vi "OpenGDS_Installer.vi"() -> ()   [LabVIEW 2020]
uses:
  OpenGDS_Installer_State.ctl
  <vilib>/Utility/config.llb/Read Key (String).vi
  <vilib>/zip/NI_Unzip.lvlib
  <vilib>/Utility/config.llb/NI_LVConfig.lvlib
panel:
  out "Tab":enum32{"Full", "Small"}(tab)
  in  "Restart":bool
  out "FullDetailsText":string
  out "FullHeader":string
  out "SmallDetailsText":string
  out "SmallHeaderText":string
  out "SmallSteps":T1(tab)
  in  "Accept":bool
  out "Lic":string
  in  "RemoveCompCode_OpenGDSSource":bool
  in  "RemoveCompCode_AddVis":bool
  out "Ready?-Text":string
  out "Status:":u8(slide) caption="Removing files" scale=0.0..100.0
  out "ProgressText":string
  in  "Back":bool
  in  "Next":bool
  in  "Cancel":bool
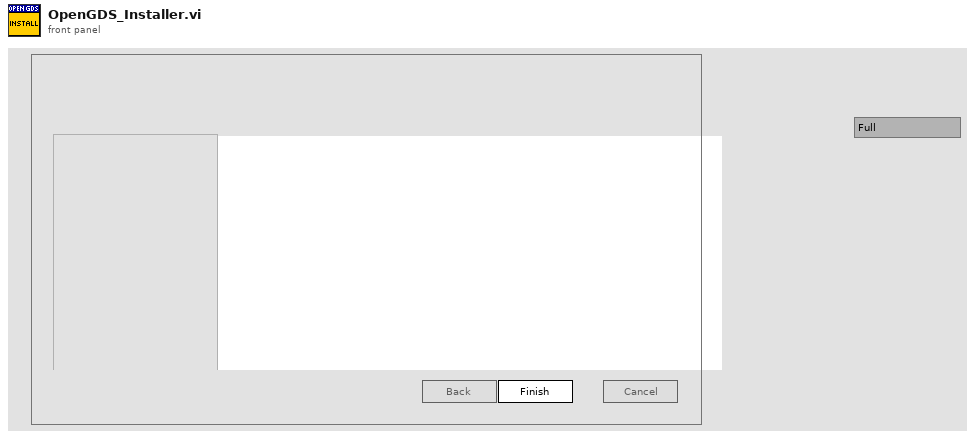
[diagram p1: front panel]
types:
  T1 = enum32{"License", "Options", "Ready?", "Progress"}
  T2 = typedef "OpenGDS_Installer_State.ctl" = enum16{"Init", "License", "Options", "Ready?", "Progress", "Cancelled", "Finished"}
  T3 = cluster{"State":T2, "FilesCopied":i32, "ErrorTest":string, "Files":path[], "ReCompile":bool, "RemoveCC":bool[]}
  T4 = typedef "LVRectTypeDef.ctl" = cluster{"Left":i16, "Top":i16, "Right":i16, "Bottom":i16}
  T5 = enum8{"Enabled", "Disabled", "Disabled and Grayed Out"}
  T6 = typedef "NI_LVConfig.lvlib/Config Data RefNum.ctl" = refnum<k1>
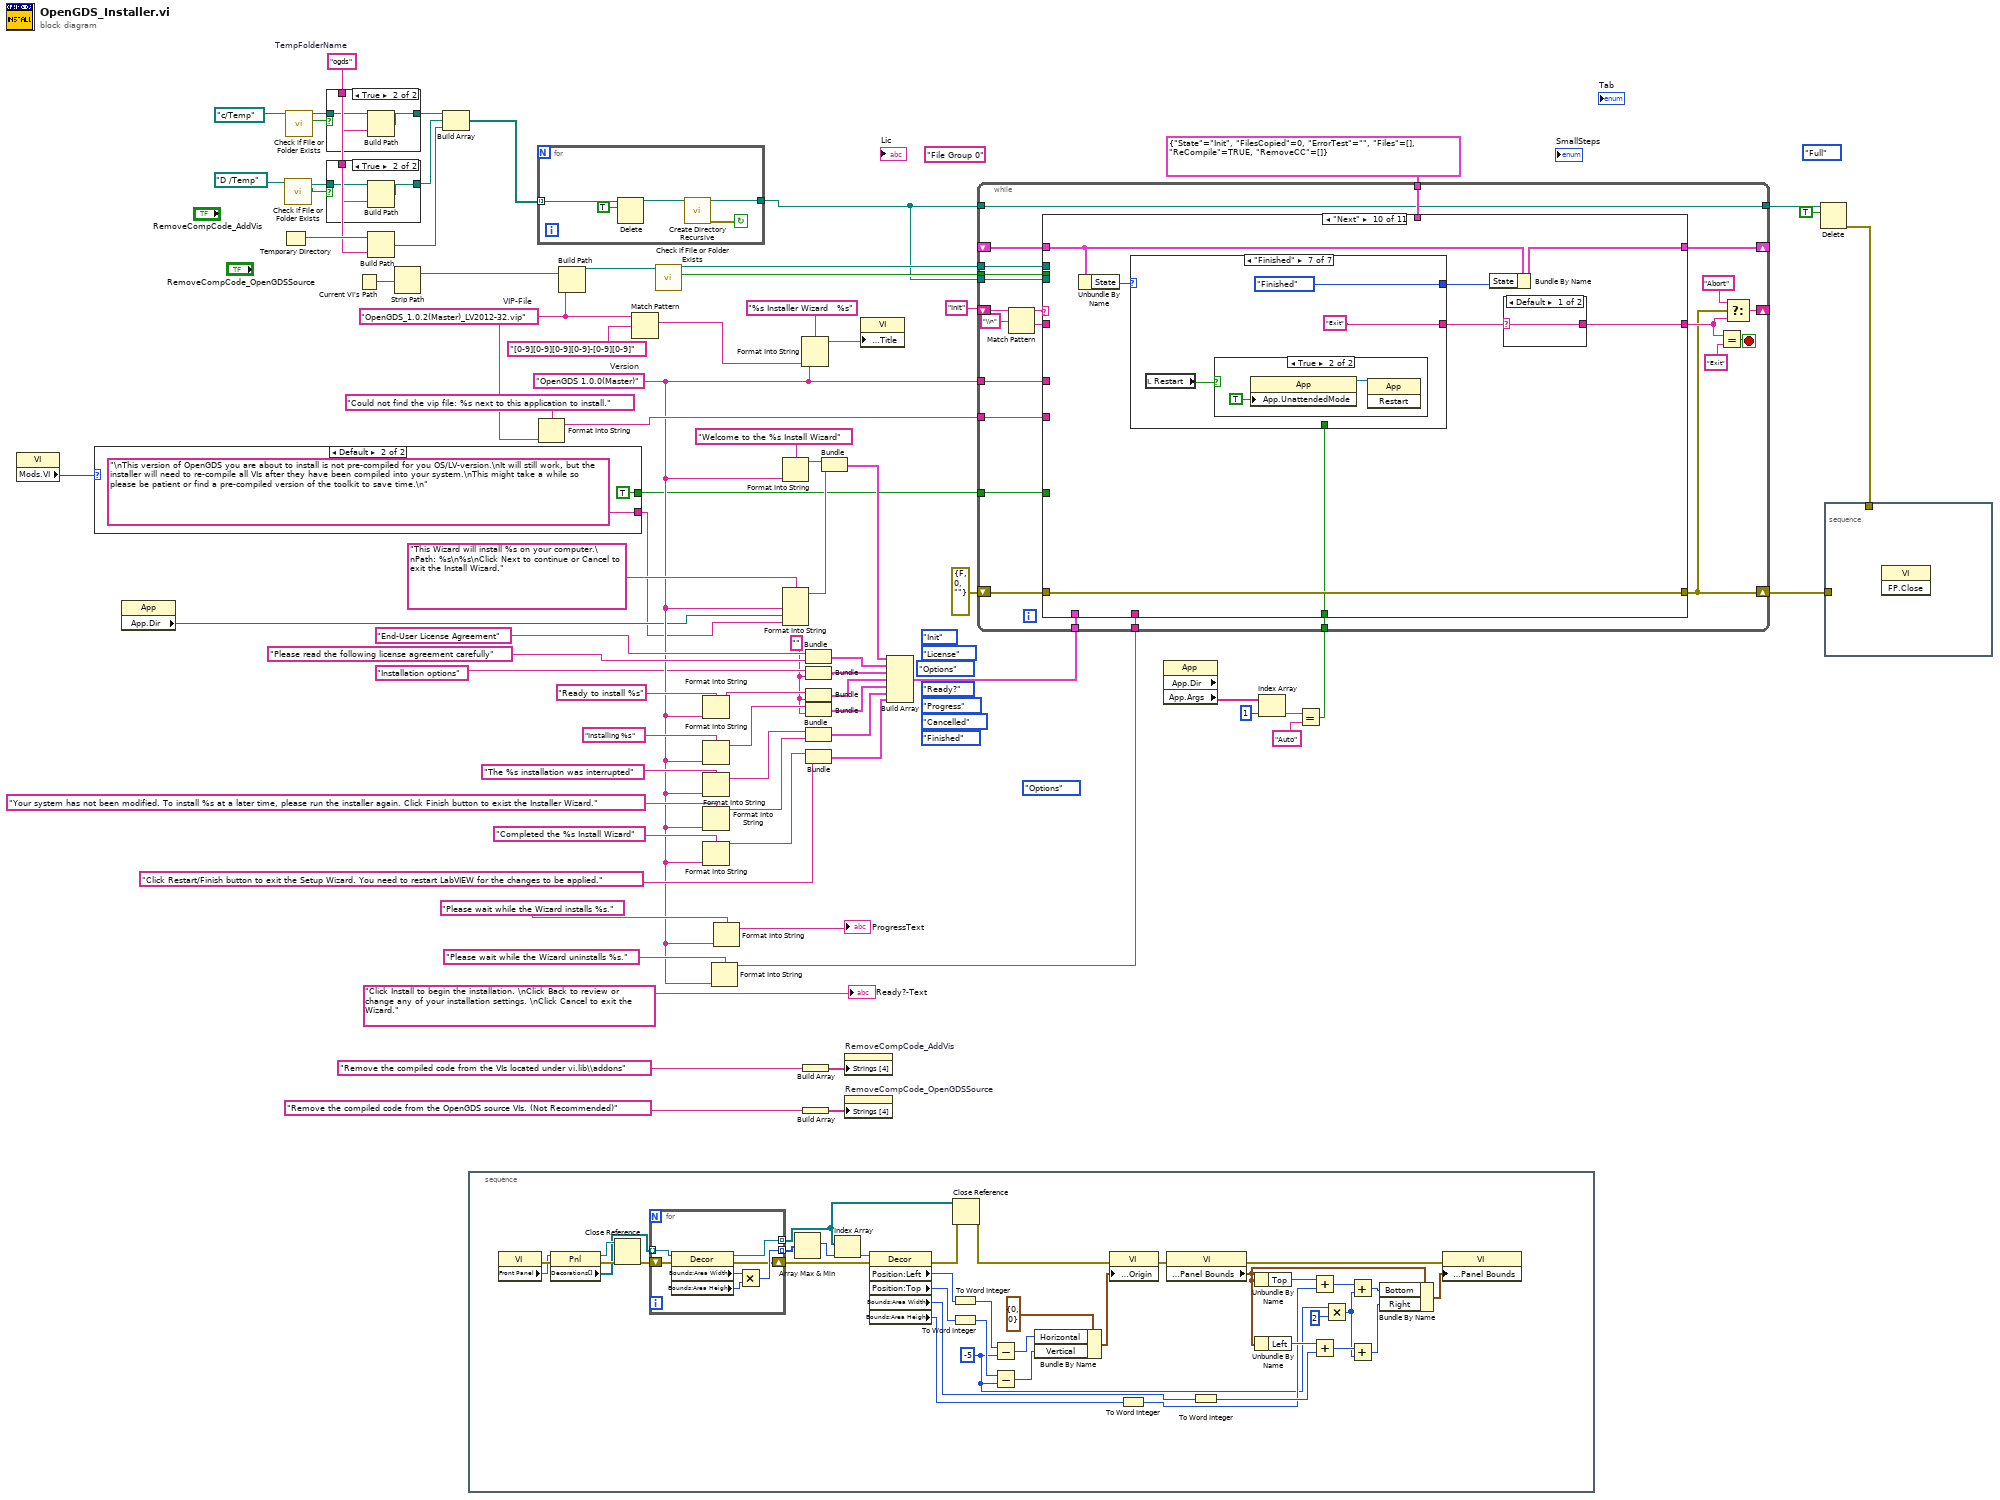
[diagram p0: block diagram]
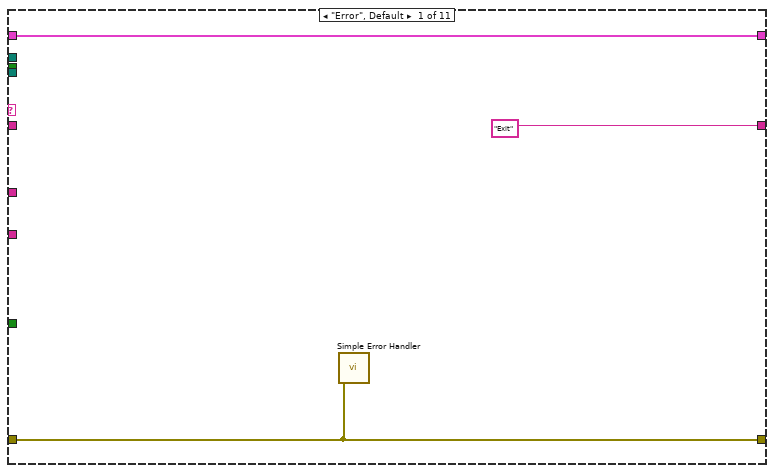
[diagram p5: hidden frame]
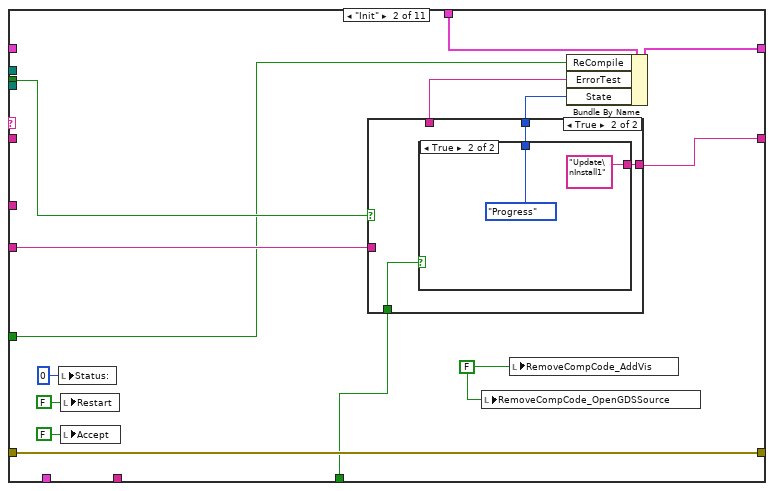
[diagram p6: hidden frame]
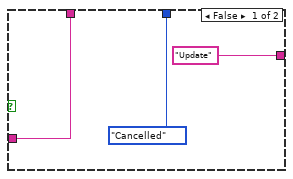
[diagram p7: hidden frame]
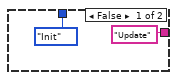
[diagram p8: hidden frame]
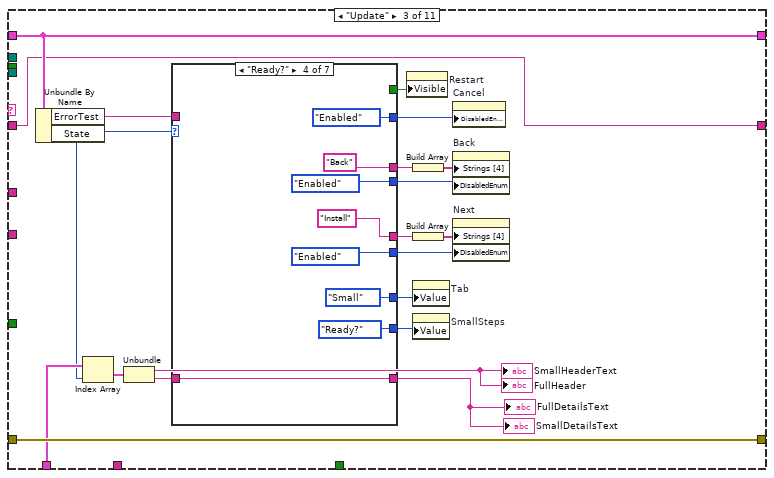
[diagram p9: hidden frame]
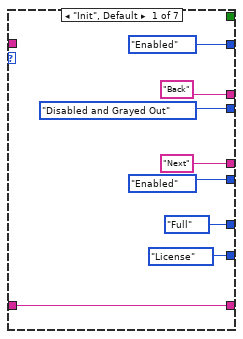
[diagram p10: hidden frame]
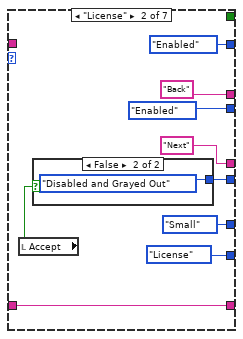
[diagram p11: hidden frame]
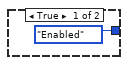
[diagram p12: hidden frame]
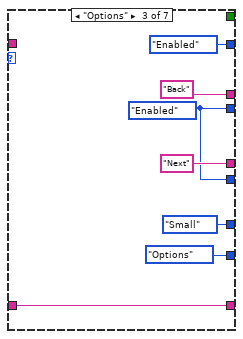
[diagram p13: hidden frame]
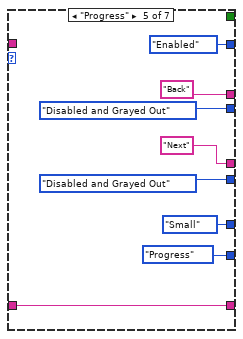
[diagram p14: hidden frame]
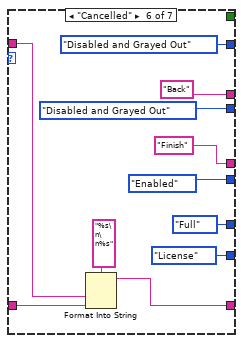
[diagram p15: hidden frame]
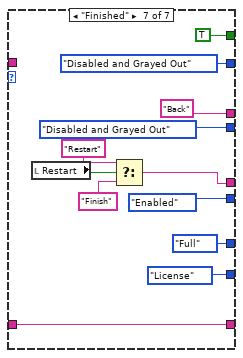
[diagram p16: hidden frame]
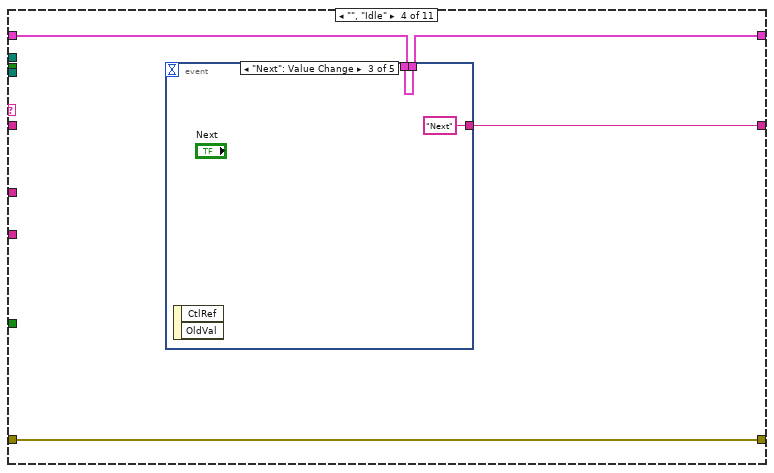
[diagram p17: hidden frame]
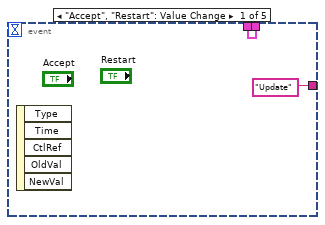
[diagram p18: hidden frame]
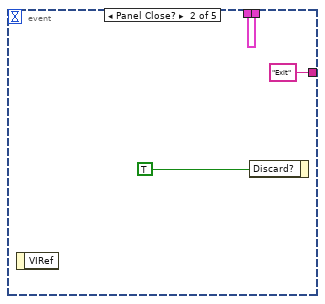
[diagram p19: hidden frame]
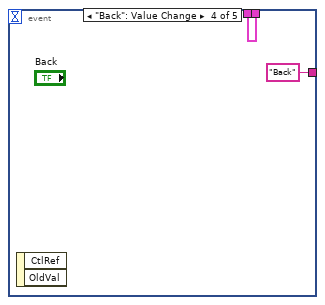
[diagram p20: hidden frame]
diagram:
  (unwired) OpenGDS_Installer_State."Options" ("State")
  (unwired) OpenGDS_Installer_State."Options" ("State")
  w17 = "ogds"  # TempFolderName
  (unwired) "File Group 0" ("section")
  w11 = "OpenGDS_1.0.2(Master)_LV2012-32.vip"  # VIP-File
  w2 = ""
  (unwired) OpenGDS_Installer_State."Finished" ("State")
  (unwired) OpenGDS_Installer_State."Cancelled" ("State")
  (unwired) OpenGDS_Installer_State."Progress" ("State")
  (unwired) OpenGDS_Installer_State."Ready?" ("State")
  (unwired) OpenGDS_Installer_State."License" ("State")
  (unwired) OpenGDS_Installer_State."Init" ("State")
  (unwired) enum32{"Full", "Small"}."Full" ("Tab")
  w40 = "OpenGDS 1.0.0(Master)"  # Version
  n1 = property class="VI"() -> ("Mods.VI"=w32:u64)  [unwired: 2 in, 2 out]
  n2 = case shown="Default" w32 {
    tunnel: [_ "\nThis version of OpenGDS you are about to install is not pre-compiled for you OS/LV-version.\nIt will still work, but the installer will need to re-compile all VIs after they have been compiled into your system.\nThis might take a while so please be patient or find a pre-compiled version of the toolkit to save time.\n"] -> w31
    tunnel: [_ TRUE] -> w30
    frame 0 {
    }
    frame Default {
    }
  }
  n3 = property class="App"() -> ("App.Dir"=w37:path)  [unwired: 2 in, 2 out]
  n4 = Temporary Directory() -> (w23:path)
  n5 = call <vilib>:"Check if File or Folder Exists.vi"("path"=path "/D /Temp") -> ("file or folder exists?"=w24:bool, "dup path"=w25:path)  [unwired: 8 in, 1 out]
  n6 = call <vilib>:"Check if File or Folder Exists.vi"("path"=path "c:/Temp") -> ("file or folder exists?"=w27:bool, "dup path"=w26:path)  [unwired: 8 in, 1 out]
  n7 = case shown="True" w27 {
    tunnel: w26 -> [w81 w84]
    tunnel: w17 -> [_ w83]
    tunnel: [w81 w82] -> w22
    frame False {
    }
    frame True {
      n8 = Build Path(base path=w84, name or relative path=w83) -> (appended path=w82:path)
    }
  }
  n9 = case shown="True" w24 {
    tunnel: w25 -> [w85 w88]
    tunnel: w17 -> [_ w87]
    tunnel: [w85 w86] -> w21
    frame False {
    }
    frame True {
      n10 = Build Path(base path=w88, name or relative path=w87) -> (appended path=w86:path)
    }
  }
  n11 = Current VI's Path() -> (path=w48:path)
  n12 = Build Path(base path=w23, name or relative path=w17) -> (appended path=w20:path)
  n13 = Strip Path(path=w48) -> (stripped path=w47:path)  [unwired: 1 out]
  n14 = Build Array(w22, w21, w20) -> (w19:path[])
  n15 = stacked-sequence {
    frame #0 {
      w92 = i16 -5 ("border spacing (2 px)")
      n16 = property on="Property Node" class="VI"() -> (error out=w125:errorcluster, "Front Panel"=w123:refnum<vi>)  [unwired: 2 in, 1 out]
      n17 = property on="Property Node" class="Pnl"(reference=w123, error in=w125) -> (reference out=w126:refnum<vi>, error out=w124:errorcluster, "Decorations[]"=w121:refnum<vi>[])
      n18 = Close Reference(reference=w126, error in (no error)=w124) -> (error out=w122:errorcluster)
      n19 = for {
        tunnel: w121 -> [w133] mode=indexing
        tunnel: [w130] -> w104 mode=indexing
        shift-right: [w128] -> w101
        shift-left: w122 -> [w129]
        tunnel: [w127] -> w91 mode=indexing
        n20 = property class="Decor"(reference=w133, error in=w129) -> (reference out=w127:refnum<vi>, error out=w128:errorcluster, "Bounds:Area Width"=w132:u32, "Bounds:Area Height"=w131:u32)
        n21 = Multiply(x=w132, y=w131) -> (x*y=w130:u32)
      }
      n22 = Array Max & Min(array=w104) -> (max index (indices)=w103:i32)  [unwired: 3 out]
      n23 = Index Array(array=w91, index=w103) -> (element=w102:refnum<vi>)
      n24 = property class="Decor"(reference=w102, error in=w101) -> (error out=w90:errorcluster, "Position:Left"=w107:i32, "Position:Top"=w110:i32, "Bounds:Area Width"=w115:u32, "Bounds:Area Height"=w113:u32)  [unwired: 1 out]
      n25 = To Word Integer(number=w107) -> (16bit integer=w94:i16)
      n26 = To Word Integer(number=w110) -> (16bit integer=w93:i16)
      n27 = Close Reference(reference=w91, error in (no error)=w90) -> (error out=w89:errorcluster)
      n28 = Subtract(x=w94, y=w92) -> (x-y=w108:i16)
      n29 = Subtract(x=w93, y=w92) -> (x-y=w109:i16)
      n30 = Bundle By Name(cluster=cluster{"Horizontal":i16, "Vertical":i16} {"Horizontal"=0, "Vertical"=0} ("Front Panel Window:Origin"), "Horizontal"=w108, "Vertical"=w109) -> (w105:cluster{"Horizontal":i16, "Vertical":i16})
      n31 = property on="Property Node" class="VI"(error in=w89, "Front Panel Window:Origin"=w105) -> (error out=w99:errorcluster)  [unwired: 1 in, 1 out]
      n32 = To Word Integer(number=w113) -> (16bit integer=w95:i16)
      n33 = property on="Property Node" class="VI"(error in=w99) -> (error out=w98:errorcluster, "Front Panel Window:Panel Bounds"=w111:T4)  [unwired: 1 in, 1 out]
      n34 = To Word Integer(number=w115) -> (16bit integer=w96:i16)
      n35 = Unbundle By Name(w111) -> ("Top"=w112:i16)
      n36 = Unbundle By Name(w111) -> ("Left"=w114:i16)
      n37 = Add(x=w112, y=w95) -> (x+y=w119:i16)
      n38 = Add(x=w114, y=w96) -> (x+y=w117:i16)
      n39 = Multiply(x=w92, y=i16 2) -> (x*y=w97:i16)
      n40 = Add(x=w119, y=w97) -> (x+y=w120:i16)
      n41 = Add(x=w117, y=w97) -> (x+y=w118:i16)
      n42 = Bundle By Name(cluster=w111, "Bottom"=w120, "Right"=w118) -> (w116:T4)
      n43 = property on="Property Node" class="VI"(error in=w98, "Front Panel Window:Panel Bounds"=w116) -> ()  [unwired: 1 in, 2 out]
    }
  }
  n44 = for {
    tunnel: [w138] -> w18
    tunnel: w19 -> [w135] mode=indexing
    stop <- w134 continue-if-true
    n45 = Delete(path (use dialog)=w135, entire hierarchy (F)=TRUE) -> (deleted path=w136:path)  [unwired: 3 in, 2 out]
    n46 = call <vilib>:"Create Directory Recursive.vi"("directory"=w136) -> ("error out"=w134:errorcluster, "directory copy"=w138:path)  [unwired: 4 in, 1 out]
  }
  n47 = Format Into String(format string="Could not find the vip file: %s next to this application to install.", w11) -> (resulting string=w42:string)  [unwired: 2 in, 1 out]
  n48 = Build Path(base path=w47, name or relative path=w11) -> (appended path=w46:path)
  n49 = Match Pattern(string=w11, regular expression="[0-9][0-9][0-9][0-9]-[0-9][0-9]") -> (match substring=w9:string)  [unwired: 1 in, 3 out]
  n50 = call <vilib>:"Check if File or Folder Exists.vi"("path"=w46) -> ("file or folder exists?"=w45:bool, "dup path"=w38:path)  [unwired: 8 in, 1 out]
  n51 = Format Into String(format string="Ready to install %s", w40) -> (resulting string=w64:string)  [unwired: 2 in, 1 out]
  n52 = Format Into String(format string="Installing %s", w40) -> (resulting string=w63:string)  [unwired: 2 in, 1 out]
  n53 = Format Into String(format string="The %s installation was interrupted", w40) -> (resulting string=w55:string)  [unwired: 2 in, 1 out]
  n54 = Format Into String(format string="Your system has not been modified. To install %s at a later time, please run the installer again. Click Finish button to exist the Installer Wizard.", w40) -> (resulting string=w54:string)  [unwired: 2 in, 1 out]
  n55 = Format Into String(format string="Completed the %s Install Wizard", w40) -> (resulting string=w58:string)  [unwired: 2 in, 1 out]
  n56 = Format Into String(format string="Please wait while the Wizard uninstalls %s." ("ProgressText"), w40) -> (resulting string=w39:string)  [unwired: 2 in, 1 out]
  n57 = Format Into String(format string="Please wait while the Wizard installs %s." ("ProgressText"), w40) -> (resulting string=→"ProgressText":string)  [unwired: 2 in, 1 out]
  n58 = Format Into String(format string="Welcome to the %s Install Wizard", w40) -> (resulting string=w69:string)  [unwired: 2 in, 1 out]
  n59 = Format Into String(format string="This Wizard will install %s on your computer.\nPath: %s\n%s\nClick Next to continue or Cancel to exit the Install Wizard.", w40, w37, w31) -> (resulting string=w68:string)  [unwired: 2 in, 1 out]
  n60 = Format Into String(format string="%s Installer Wizard   %s", w40, w9) -> (resulting string=w75:string)  [unwired: 2 in, 1 out]
  n61 = Build Array("Remove the compiled code from the VIs located under vi.lib\\addons" ("ProgressText")) -> (w8:string[])
  n62 = Build Array("Remove the compiled code from the OpenGDS source VIs. (Not Recommended)" ("ProgressText")) -> (w6:string[])
  n63 = Bundle("End-User License Agreement", "Please read the following license agreement carefully") -> (w66:cluster{string, string})  [unwired: 1 in]
  n64 = Bundle("Installation options", w2) -> (w1:cluster{string, string})  [unwired: 1 in]
  n65 = Bundle(w64, w2) -> (w4:cluster{string, string})  [unwired: 1 in]
  n66 = Bundle(w63, w2) -> (w62:cluster{string, string})  [unwired: 1 in]
  n67 = Bundle(w55, w54) -> (w61:cluster{string, string})  [unwired: 1 in]
  n68 = Bundle(w58, "input 1"="Click Restart/Finish button to exit the Setup Wizard. You need to restart LabVIEW for the changes to be applied.") -> (w60:cluster{string, "input 1":string})  [unwired: 1 in]
  n69 = Bundle(w69, w68) -> (w67:cluster{string, string})  [unwired: 1 in]
  n70 = property on="RemoveCompCode_AddVis" class="Bool (strict)"("Strings [4]"=w8) -> ()  [unwired: 2 in, 2 out]
  n71 = property on="RemoveCompCode_OpenGDSSource" class="Bool (strict)"("Strings [4]"=w6) -> ()  [unwired: 2 in, 2 out]
  n72 = property on="Property Node" class="VI"("Front Panel.Title"=w75) -> ()  [unwired: 2 in, 2 out]
  n73 = Build Array(w67, w66, w1, w4, w62, w61, w60) -> (w70:cluster{string, "input 1":string}[])
  n74 = property class="App" props=["App.Dir", "App.Args"]() -> ("App.Args"=w13:string[])  [unwired: 2 in, 3 out]
  n75 = Index Array(array=w13, index=1) -> (element=w15:string)
  n76 = Equal?(x=w15, y="Auto") -> (x = y?=w12:bool)
  n77 = while {
    shift-right: [w156] -> w34
    shift-left: errorcluster {"status"=FALSE, "code"=0, "source"=""} ("error IO") -> [w162]
    shift-right: [w161] -> _
    shift-left: "Init" -> [w152]
    shift-right: [w155] -> _
    shift-left: _ -> [w154]
    tunnel: w40 -> [w153]
    tunnel: w70 -> [w148]
    tunnel: w45 -> [w147]
    tunnel: w42 -> [w146]
    tunnel: T3 {"State"=enum."Init", "FilesCopied"=0, "ErrorTest"="", "Files"=[], "ReCompile"=TRUE, "RemoveCC"=[]} -> [w145]
    tunnel: w39 -> [w144]
    tunnel: w38 -> [w143]
    tunnel: w18 -> [w142]
    tunnel: w18 -> [w141]
    tunnel: [w141] -> w36
    tunnel: w30 -> [w140]
    tunnel: w12 -> [w139]
    stop <- w160 stop-if-true
    n78 = Match Pattern(string=w152, regular expression="\\n") -> (before substring=w151:string, after substring=w149:string)  [unwired: 1 in, 2 out]
    n79 = case shown="\"Next\"" w151 {
      tunnel: w162 -> [w163 w179 w208 w275 w306 w327 w372 w438 w543 w557 w580]
      tunnel: [w163 w179 w208 w275 w293 w333 w371 w435 w543 w557 w580] -> w156
      tunnel: ["Exit" w168 w201 w276 "Update" w344 w379 w449 "Next" w558 w581] -> w157
      tunnel: [w164 w178 w209 w277 w302 w345 w381 w436 w545 w561 w584] -> w155
      tunnel: w154 -> [w164 _ w209 w278 w300 w346 w362 w436 w545 w562 w585]
      tunnel: w153 -> [_ _ _ _ _ _ _ _ _ _ _]
      tunnel: w149 -> [_ _ w201 _ _ _ _ _ _ _ _]
      tunnel: w148 -> [_ _ w197 _ _ _ _ _ _ _ _]
      tunnel: w147 -> [_ w175 _ _ _ _ _ _ _ _ _]
      tunnel: w146 -> [_ w174 _ _ _ _ _ _ _ _ _]
      tunnel: w145 -> [_ w172 _ _ _ _ _ _ _ _ _]
      tunnel: w144 -> [_ _ _ _ w298 _ _ _ _ _ _]
      tunnel: w143 -> [_ _ _ _ _ w343 _ _ _ _ _]
      tunnel: w142 -> [_ _ _ _ _ w338 w377 _ _ _ _]
      tunnel: w140 -> [_ w169 _ _ _ _ _ _ _ _ _]
      tunnel: w139 -> [_ w167 _ _ _ _ _ _ _ w555 _]
      frame "Error", Default {
        n80 = call <vilib>:"Simple Error Handler.vi"("error in (no error)"=w163) -> ()  [unwired: 4 in, 5 out]
      }
      frame "Init" {
        w166 = FALSE ("Restart")
        n81 = local write "Status:"(u8 0 ("Status:")) -> ()
        n82 = local write "Restart"(FALSE ("Restart")) -> ()
        n83 = local write "Accept"(FALSE ("Accept")) -> ()
        n84 = case shown="True" w175 {
          tunnel: w174 -> [w181 _]
          tunnel: [OpenGDS_Installer_State."Cancelled" ("State") w185] -> w173
          tunnel: [w181 _] -> w171
          tunnel: ["Update" w184] -> w168
          tunnel: w167 -> [_ w183]
          frame False {
          }
          frame True {
            n85 = case shown="True" w183 {
              tunnel: [OpenGDS_Installer_State."Init" ("State") OpenGDS_Installer_State."Progress" ("State")] -> w185
              tunnel: ["Update" "Update\nInstall1"] -> w184
              frame False {
              }
              frame True {
              }
            }
          }
        }
        n86 = local write "RemoveCompCode_OpenGDSSource"(w166) -> ()
        n87 = local write "RemoveCompCode_AddVis"(w166) -> ()
        n88 = Bundle By Name(cluster=w172, "ReCompile"=w169, "ErrorTest"=w171, "State"=w173) -> (w178:T3)
      }
      frame "Update" {
        n89 = Unbundle By Name(w209) -> ("ErrorTest"=w190:string, "State"=w196:T2)
        n90 = Index Array(array=w197, index=w196) -> (element=w194:cluster{string, "input 1":string})
        n91 = Unbundle(w194) -> (→"SmallHeaderText" →"FullHeader":string, "input 1"=w192:string)
        n92 = case shown="\"Ready?\"" w196 {
          tunnel: ["Back" "Back" "Back" "Back" "Back" "Back" "Back"] -> w205
          tunnel: ["Next" "Next" "Next" "Install" "Next" "Finish" w265] -> w204
          tunnel: [T5."Enabled" ("Disabled") w224 w230 T5."Enabled" ("Disabled") T5."Disabled and Grayed Out" ("Disabled") T5."Enabled" ("Disabled") T5."Enabled" ("Disabled")] -> w203
          tunnel: [T5."Disabled and Grayed Out" ("Disabled") T5."Enabled" ("Disabled") w230 T5."Enabled" ("Disabled") T5."Disabled and Grayed Out" ("Disabled") T5."Disabled and Grayed Out" ("Disabled") T5."Disabled and Grayed Out" ("Disabled")] -> w202
          tunnel: [enum32{"Full", "Small"}."Full" ("Tab") enum32{"Full", "Small"}."Small" ("Tab") enum32{"Full", "Small"}."Small" ("Tab") enum32{"Full", "Small"}."Small" ("Tab") enum32{"Full", "Small"}."Small" ("Tab") enum32{"Full", "Small"}."Full" ("Tab") enum32{"Full", "Small"}."Full" ("Tab")] -> w200
          tunnel: [T1."License" ("SmallSteps") T1."License" ("SmallSteps") T1."Options" ("SmallSteps") T1."Ready?" ("SmallSteps") T1."Progress" ("SmallSteps") T1."License" ("SmallSteps") T1."License" ("SmallSteps")] -> w199
          tunnel: [T5."Enabled" ("Disabled") T5."Enabled" ("Disabled") T5."Enabled" ("Disabled") T5."Enabled" ("Disabled") T5."Enabled" ("Disabled") T5."Disabled and Grayed Out" ("Disabled") T5."Disabled and Grayed Out" ("Disabled")] -> w198
          tunnel: [_ _ _ _ _ _ TRUE] -> w195
          tunnel: w192 -> [w211 w219 w231 w237 w245 w256 w264]
          tunnel: [w211 w219 w231 w237 w245 w255 w264] -> w191
          tunnel: w190 -> [_ _ _ _ _ w253 _]
          frame "Init", Default {
          }
          frame "License" {
            n93 = local read "Accept"() -> (w222:bool)
            n94 = case shown="False" w222 {
              tunnel: [T5."Enabled" ("Disabled") T5."Disabled and Grayed Out" ("Disabled")] -> w224
              frame True {
              }
              frame False {
              }
            }
          }
          frame "Options" {
            w230 = T5."Enabled" ("Disabled")
          }
          frame "Ready?" {
          }
          frame "Progress" {
          }
          frame "Cancelled" {
            n95 = Format Into String(format string="%s\n\n%s", w253, w256) -> (resulting string=w255:string)  [unwired: 2 in, 1 out]
          }
          frame "Finished" {
            n96 = local read "Restart"() -> (w268:bool)
            n97 = Select(t="Restart", s=w268, f="Finish") -> (s? t:f=w265:string)
          }
        }
        "FullDetailsText" <- w191
        "SmallDetailsText" <- w191
        n98 = property on="Restart" class="Bool (strict)"("Visible"=w195) -> ()  [unwired: 2 in, 2 out]
        n99 = Build Array(w205) -> (w207:string[])
        n100 = Build Array(w204) -> (w206:string[])
        n101 = property on="Tab" class="TabCtl (strict)"("Value"=w200) -> ()  [unwired: 2 in, 2 out]
        n102 = property on="SmallSteps" class="TabCtl (strict)"("Value"=w199) -> ()  [unwired: 2 in, 2 out]
        n103 = property on="Cancel" class="Bool (strict)"("DisabledEnum"=w198) -> ()  [unwired: 2 in, 2 out]
        n104 = property on="Back" class="Bool"("Strings [4]"=w207, "DisabledEnum"=w202) -> ()  [unwired: 2 in, 2 out]
        n105 = property on="Next" class="Bool"("Strings [4]"=w206, "DisabledEnum"=w203) -> ()  [unwired: 2 in, 2 out]
      }
      frame "", "Idle" {
        n106 = event shown="[2] \"Next\": Value Change" {
          selector: _ -> [_ _ _ _ _]
          dyn-events: _ -> [_ _ _ _ _]
          timeout: _ -> [_ _ _ _ _]
          tunnel: w278 -> [w280 w282 w285 w287 w292]
          tunnel: [w280 w282 w285 w287 w289] -> w277
          tunnel: ["Update" "Exit" "Next" "Back" "Update\nAbort"] -> w276
          event "Accept", "Restart": Value Change {
            n107 = event-data() -> ()  [unwired: 1 in, 5 out]
          }
          event Panel Close? {
            n108 = event-data() -> ()  [unwired: 1 in, 1 out]
            n109 = event-data("Discard?"=TRUE) -> ()  [unwired: 1 in, 1 out]
          }
          event "Next": Value Change {
            n110 = event-data() -> ()  [unwired: 1 in, 2 out]
          }
          event "Back": Value Change {
            n111 = event-data() -> ()  [unwired: 1 in, 2 out]
          }
          event "Cancel": Value Change {
            n112 = event-data() -> ()  [unwired: 1 in, 2 out]
            n113 = Bundle By Name(cluster=w292, "State"=OpenGDS_Installer_State."Cancelled") -> (w289:T3)
            n114 = local write "Cancel"(FALSE ("Cancel")) -> ()
          }
        }
      }
      frame "Abort" {
        # "Remove Files"
        n115 = Unbundle By Name(w300) -> ("Files"=w296:path[], "FilesCopied"=w297:i32)
        n116 = property class="App"() -> ("App.Dir"=w294:path)  [unwired: 2 in, 2 out]
        n117 = local write "Cancel"(FALSE ("Cancel")) -> ()
        n118 = Array Size(array=w296) -> (size(s)=w295:i32)
        n119 = for {
          N: w297 -> [w313]
          tunnel: w296 -> [w312] mode=indexing
          tunnel: w295 -> [w314]
          tunnel: w294 -> [w311]
          i -> [w317]
          n120 = Build Path(base path=w311, name or relative path=w312) -> (appended path=w307:path)
          n121 = Subtract(x=w313, y=w317) -> (x-y=w315:i32)
          n122 = Increment(x=w315) -> (x+1=w318:i32)
          n123 = Path To String(path=w307) -> (string=w309:string)
          n124 = Divide(x=w318, y=w314) -> (x/y=w320:dbl)
          n125 = Match Pattern(string=w309, regular expression="addons") -> (offset past match=w308:i32)  [unwired: 1 in, 3 out]
          n126 = Multiply(x=w320, y=100.0) -> (x*y=w316:dbl)
          n127 = local write "Status:"(w316) -> ()
          n128 = case shown="-1" w308 {
            tunnel: w307 -> [_ w321]
            frame 0, Default {
            }
            frame -1 {
              n129 = Set Permissions(7:i16 511 ("permissions"), 11:w321) -> (0:w323:errorcluster, 3:w322:path)  [unwired: 3 in]
              n130 = Delete(path (use dialog)=w322, error in=w323) -> ()  [unwired: 3 in, 3 out]
            }
          }
        }
        n131 = local write "ProgressText"(w298) -> ()
        n132 = Bundle By Name(cluster=w300, "State"=OpenGDS_Installer_State."Cancelled") -> (w302:T3)
        n133 = property on="Cancel" class="Bool (strict)"("DisabledEnum"=T5."Disabled and Grayed Out" ("Disabled")) -> ()  [unwired: 2 in, 2 out]
        n134 = property on="Status:" class="Slide (strict)"("Caption.Text"="Removing files") -> ()  [unwired: 2 in, 2 out]
        n135 = call <vilib>:"Clear Errors.vi"("error in (no error)"=w306) -> ("error out"=w293:errorcluster)  [unwired: 5 in, 1 out]
      }
      frame "Install1" {
        n136 = property on="Status:" class="Slide (strict)"(error in=w327, "Caption.Text"="Unzipping Files") -> (error out=w326:errorcluster)  [unwired: 1 in, 1 out]
        n137 = call <vilib>:"Unzip.vi"("error in (no error)"=w326, "Target directory (same as Zip file if empty)"=w338, "Zip file"=w343) -> ("error out"=w335:errorcluster)  [unwired: 6 in, 2 out]
        n138 = Build Path(base path=w338, name or relative path="spec") -> (appended path=w336:path)
        n139 = local write "Status:"(u8 0 ("Status:")) -> ()
        n140 = call <vilib>:"Open Config Data.vi"("error in (no error)"=w335, "create file if necessary (T)"=FALSE, "configuration file path"=w336) -> ("error out"=w340:errorcluster, "refnum"=w342:T6)  [unwired: 6 in, 1 out]
        n141 = while {
          shift-right: [w351] -> w341
          shift-left: w340 -> [w358]
          tunnel: w342 -> [w357]
          tunnel: [w347] -> w334 mode=indexing if=w352
          tunnel: [w349] -> w332
          i -> [w356]
          stop <- w350 continue-if-true
          n142 = Format Into String(format string="File %d", w356) -> (resulting string=w354:string)  [unwired: 2 in, 1 out]
          n143 = local read "Cancel"() -> (w349:bool)
          n144 = call-poly <vilib>:"Read Key.vi"("section"="File Group 0", "error in (no error)"=w358, "key"=w354, "refnum"=w357) -> ("error out"=w351:errorcluster, "value"=w348:string, "found?"=w352:bool)  [unwired: 4 in, 1 out]
          n145 = String To Path(string=w348) -> (path=w347:path)
          n146 = Compound Arithmetic op=AND(w352, invert w351, invert w349) -> (w350:bool)
        }
        n147 = call <vilib>:"Close Config Data.vi"("error in (no error)"=w341, "refnum"=w342) -> ("error out"=w333:errorcluster)  [unwired: 8 in, 1 out]
        n148 = Bundle By Name(cluster=w346, "FilesCopied"=0, "Files"=w334) -> (w345:T3)
        n149 = Select(t="Abort", s=w332, f="Install2") -> (s? t:f=w344:string)
      }
      frame "Install2" {
        n150 = local read "RemoveCompCode_OpenGDSSource"() -> (w361:bool)
        n151 = local read "RemoveCompCode_AddVis"() -> (w360:bool)
        n152 = Build Path(base path=w377, name or relative path="File Group 0" ("section")) -> (appended path=w375:path)
        n153 = property class="App"() -> ("App.Dir"=w373:path)  [unwired: 2 in, 2 out]
        n154 = property on="Status:" class="Slide (strict)"("Caption.Text"="Copying files") -> ()  [unwired: 2 in, 2 out]
        n155 = Unbundle By Name(w362) -> ("Files"=w374:path[])
        n156 = Unbundle By Name(w362) -> ("ReCompile"=w366:bool)
        n157 = for {
          N -> [w411]
          shift-right: [w402] -> w371
          shift-left: w372 -> [w418]
          tunnel: w375 -> [w406]
          tunnel: w374 -> [w404] mode=indexing
          tunnel: w373 -> [w405]
          tunnel: [w401] -> w364
          tunnel: [w398] -> w370
          tunnel: w366 -> [w390]
          tunnel: [w397] -> w365 mode=indexing
          tunnel: w361 -> [w387]
          tunnel: w360 -> [w385]
          tunnel: [w382] -> w359 mode=indexing
          i -> [w400]
          stop <- w399 stop-if-true
          n158 = Build Path(base path=w405, name or relative path=w404) -> (appended path=w403:path)
          n159 = Build Path(base path=w406, name or relative path=w404) -> (appended path=w396:path)
          n160 = Path To String(path=w396) -> (string=w392:string)
          n161 = Strip Path(path=w403) -> (stripped path=w419:path)  [unwired: 1 out]
          n162 = Increment(x=w400) -> (x+1=w398:i32)
          n163 = Match Pattern(string=w392, regular expression="[\\\\/]Providers[\\\\/]") -> (offset past match=w394:i32)  [unwired: 1 in, 3 out]
          n164 = Match Pattern(string=w392, regular expression="[\\\\/]addons[\\\\/]") -> (offset past match=w393:i32)  [unwired: 1 in, 3 out]
          n165 = call <vilib>:"Create Directory Recursive.vi"("error in (no error)"=w418, "directory"=w419) -> ("error out"=w417:errorcluster)  [unwired: 3 in, 2 out]
          n166 = Divide(x=w398, y=w411) -> (x/y=w410:dbl)
          n167 = Greater Or Equal To 0?(x=w394) -> (x >= 0?=w388:bool)
          n168 = Greater Or Equal To 0?(x=w393) -> (x >= 0?=w386:bool)
          n169 = call <vilib>:"Check if File or Folder Exists.vi"("error in (no error)"=w417, "path"=w403) -> ("error out"=w416:errorcluster, "file or folder exists?"=w413:bool, "dup path"=w415:path)  [unwired: 7 in]
          n170 = Compound Arithmetic op=AND(w387, w388) -> (w384:bool)
          n171 = Compound Arithmetic op=AND(w385, w386) -> (w383:bool)
          n172 = Multiply(x=w410, y=100.0) -> (x*y=→"Status:":dbl)
          n173 = case shown="True" w413 {
            tunnel: w416 -> [w425 w429]
            tunnel: w415 -> [_ w428]
            tunnel: [w425 w426] -> w414
            frame False {
            }
            frame True {
              n174 = Set Permissions(7:i16 511 ("permissions"), 8:w429, 11:w428) -> (0:w426:errorcluster)  [unwired: 2 in, 1 out]
            }
          }
          n175 = Compound Arithmetic op=OR(w390, w384, w383) -> (w389:bool)
          n176 = local read "Cancel"() -> (w401:bool)
          n177 = Copy(8:w414, 9:TRUE ("overwrite (F)"), 10:w403, 11:w396) -> (0:w408:errorcluster, 3:w397:path)  [unwired: 1 in, 1 out]
          n178 = case shown="True" w389 {
            tunnel: w397 -> [w422 _]
            tunnel: w408 -> [w421 w424]
            tunnel: [w420 w424] -> w402
            frame False {
              n179 = Set Permissions(7:i16 365 ("permissions"), 8:w421, 11:w422) -> (0:w420:errorcluster)  [unwired: 2 in, 1 out]
            }
            frame True {
            }
          }
          n180 = Or(x=w384, y=w383) -> (x .or. y?=w382:bool)
          n181 = Or(x=w402, y=w401) -> (x .or. y?=w399:bool)
        }
        n182 = Compound Arithmetic op=OR(w366, w360, w361) -> (w363:bool)
        n183 = Bundle By Name(cluster=w362, "FilesCopied"=w370, "Files"=w365, "RemoveCC"=w359) -> (w381:T3)
        n184 = Select(t="ReCompile1", s=w363, f="Next") -> (s? t:f=w368:string)
        n185 = Select(t="Abort", s=w364, f=w368) -> (s? t:f=w379:string)
      }
      frame "ReCompile1" {
        n186 = Unbundle By Name(w436) -> ("RemoveCC"=w432:bool[], "ReCompile"=w430:bool, "Files"=w437:path[])
        n187 = property on="Status:" class="Slide (strict)"("Caption.Text"="Re-compiling") -> (error out=w431:errorcluster)  [unwired: 2 in, 1 out]
        n188 = for {
          N -> [w476]
          tunnel: [w488] -> w433 mode=concatenating if=w487
          shift-right: [w474] -> w439
          shift-left: w438 -> [w481]
          tunnel: [w486] -> w444 mode=indexing if=w485
          tunnel: [w484] -> w445 mode=indexing if=w483
          tunnel: w437 -> [w472] mode=indexing
          tunnel: [w471] -> w434
          tunnel: w432 -> [w469] mode=indexing
          tunnel: w431 -> [_]
          tunnel: w430 -> [w468]
          i -> [w477]
          stop <- w473 stop-if-true
          n189 = call <vilib>:"Get File Extension.vi"("error in (no error)"=w481, "file"=w472) -> ("error out"=w482:errorcluster, "lowercase file extension"=w490:string, "dup file"=w489:path)  [unwired: 5 in, 2 out]
          n190 = Or(x=w469, y=w468) -> (x .or. y?=w470:bool)
          n191 = case shown="True" w470 {
            tunnel: w490 -> [_ w502]
            tunnel: w489 -> [_ w501]
            tunnel: [_ w500] -> w488
            tunnel: [_ w499] -> w487
            tunnel: [_ w498] -> w486
            tunnel: [_ w497] -> w485
            tunnel: [_ w496] -> w484
            tunnel: [_ w495] -> w483
            tunnel: w482 -> [w491 w494]
            tunnel: [w491 w493] -> w474
            tunnel: w469 -> [_ w492]
            frame False {
            }
            frame True {
              n192 = case shown="\"llb\"" w502 {
                tunnel: w494 -> [w503 w511 w518 w523 w526]
                tunnel: w501 -> [_ w510 w517 w522 w525]
                tunnel: [_ w508 _ _ w531] -> w500
                tunnel: [_ TRUE _ _ TRUE] -> w499
                tunnel: [w503 w506 w516 w519 w529] -> w493
                tunnel: [_ _ _ w521 _] -> w498
                tunnel: [_ _ _ TRUE _] -> w497
                tunnel: [_ _ w515 _ _] -> w496
                tunnel: [_ _ TRUE _ _] -> w495
                tunnel: w492 -> [_ w504 _ _ w524]
                frame Default {
                }
                frame "ctl", "vi", "vit" {
                  n193 = Open VI Reference(vi path=w510, options=2, error in (no error)=w511) -> (vi reference=w505:refnum<vi>, error out=w506:errorcluster)  [unwired: 3 in]
                  n194 = case shown="True" w504 {
                    tunnel: w505 -> [_ w513]
                    frame False {
                    }
                    frame True {
                      n195 = property class="VI"(reference=w513, "ContainstCompiledCode"=FALSE ("Contains Compiled Code")) -> ()  [unwired: 1 in, 2 out]
                    }
                  }
                  n196 = Build Array(w505) -> (w508:refnum<vi>[])
                }
                frame "lvclass" {
                  n197 = invoke class="App" method="LVClass.Open"(error in=w518, "Path"=w517) -> (error out=w516:errorcluster, "LVClass.Open"=w515:refnum<vi>)  [unwired: 2 in, 2 out]
                }
                frame "lvlib" {
                  n198 = invoke class="App" method="Library.Open"(error in=w523, "path"=w522) -> (error out=w519:errorcluster, "Open Library"=w521:refnum<vi>)  [unwired: 2 in, 2 out]
                }
                frame "llb" {
                  n199 = List Folder(path=w525, error in=w526) -> (filenames=w527:string[], error out=w528:errorcluster)  [unwired: 1 in, 3 out]
                  n200 = for {
                    tunnel: w527 -> [w535] mode=indexing
                    tunnel: w525 -> [w539]
                    shift-right: [w536] -> w529
                    shift-left: w528 -> [w537]
                    tunnel: [w532] -> w531 mode=indexing
                    tunnel: w524 -> [w533]
                    n201 = Build Path(base path=w539, name or relative path=w535) -> (appended path=w538:path)
                    n202 = Open VI Reference(vi path=w538, options=2, error in (no error)=w537) -> (vi reference=w532:refnum<vi>, error out=w536:errorcluster)  [unwired: 3 in]
                    n203 = case shown="True" w533 {
                      tunnel: w532 -> [_ w541]
                      frame False {
                      }
                      frame True {
                        n204 = property class="VI"(reference=w541, "ContainstCompiledCode"=FALSE ("Contains Compiled Code")) -> ()  [unwired: 1 in, 2 out]
                      }
                    }
                  }
                }
              }
            }
          }
          n205 = Increment(x=w477) -> (x+1=w479:i32)
          n206 = Divide(x=w479, y=w476) -> (x/y=w478:dbl)
          n207 = Multiply(x=w478, y=20.0) -> (x*y=w480:dbl)
          n208 = local write "Status:"(w480) -> ()
          n209 = local read "Cancel"() -> (w471:bool)
          n210 = Or(x=w474, y=w471) -> (x .or. y?=w473:bool)
        }
        n211 = for {
          N -> [w461]
          tunnel: w433 -> [w467] mode=indexing
          shift-right: [w465] -> w440
          shift-left: w439 -> [w466]
          i -> [w460]
          n212 = invoke class="VI" method="Save.Instrument"(reference=w467, error in=w466) -> (error out=w465:errorcluster)  [unwired: 4 in, 5 out]
          n213 = Increment(x=w460) -> (x+1=w462:i32)
          n214 = Divide(x=w462, y=w461) -> (x/y=w463:dbl)
          n215 = Multiply(x=w463, y=80.0) -> (x*y=w459:dbl)
          n216 = Add(x=w459, y=20.0) -> (x+y=w457:dbl)
          n217 = local write "Status:"(w457) -> ()
        }
        n218 = for {
          tunnel: w444 -> [w456] mode=indexing
          shift-right: [w454] -> w441
          shift-left: w440 -> [w455]
          n219 = invoke class="Library" method="Save"(reference=w456, error in=w455) -> (error out=w454:errorcluster)  [unwired: 2 in, 3 out]
        }
        n220 = for {
          tunnel: w445 -> [w453] mode=indexing
          shift-right: [w451] -> w442
          shift-left: w441 -> [w452]
          n221 = invoke class="LVClassLibrary" method="Save"(reference=w453, error in=w452) -> (error out=w451:errorcluster)  [unwired: 2 in, 3 out]
        }
        n222 = Close Reference(reference=w433, error in (no error)=w442) -> (error out=w443:errorcluster)
        n223 = Close Reference(reference=w444, error in (no error)=w443) -> (error out=w446:errorcluster)
        n224 = Close Reference(reference=w445, error in (no error)=w446) -> (error out=w435:errorcluster)
        n225 = Select(t="Abort", s=w434, f="ReCompile2") -> (s? t:f=w449:string)
      }
      frame "ReCompile2" {
        n226 = Unbundle By Name(w545) -> ("Files"=w546:path[])
        n227 = for {
          N -> [w547]
          tunnel: w546 -> [w553] mode=indexing
          i -> [w548]
          n228 = Increment(x=w548) -> (x+1=w551:i32)
          n229 = Set Permissions(7:i16 365 ("permissions"), 11:w553) -> ()  [unwired: 3 in, 2 out]
          n230 = Divide(x=w551, y=w547) -> (x/y=w550:dbl)
          n231 = Multiply(x=w550, y=100.0) -> (x*y=w552:dbl)
          n232 = local write "Status:"(w552) -> ()
        }
        n233 = property on="Status:" class="Slide (strict)"("Caption.Text"="Setting file permissions") -> ()  [unwired: 2 in, 2 out]
      }
      frame "Next" {
        n234 = Unbundle By Name(w562) -> ("State"=w560:T2)
        n235 = case shown="\"Finished\"" w560 {
          tunnel: [OpenGDS_Installer_State."License" ("State") OpenGDS_Installer_State."Options" ("State") OpenGDS_Installer_State."Ready?" ("State") OpenGDS_Installer_State."Progress" ("State") OpenGDS_Installer_State."Finished" ("State") OpenGDS_Installer_State."Cancelled" ("State") OpenGDS_Installer_State."Finished" ("State")] -> w559
          tunnel: [_ _ _ "Update\nInstall1" _ "Exit" "Exit"] -> w556
          tunnel: w555 -> [_ _ _ _ w570 _ _]
          frame "Init", Default {
          }
          frame "License" {
          }
          frame "Options" {
          }
          frame "Ready?" {
          }
          frame "Progress" {
            n236 = case shown="True" w570 {
              frame False {
              }
              frame True {
                n237 = Quit LabVIEW() -> ()  [unwired: 1 in]
              }
            }
          }
          frame "Cancelled" {
          }
          frame "Finished" {
            n238 = local read "Restart"() -> (w574:bool)
            n239 = case shown="True" w574 {
              frame False {
              }
              frame True {
                n240 = property class="App"("App.UnattendedMode"=TRUE ("Application:Unattended Mode")) -> (reference out=w577:refnum<vi>)  [unwired: 2 in, 1 out]
                n241 = invoke class="App" method="Restart"(reference=w577) -> ()  [unwired: 2 in, 3 out]
              }
            }
          }
        }
        n242 = Bundle By Name(cluster=w562, "State"=w559) -> (w561:T3)
        n243 = case shown="Default" w556 {
          selector: w556 -> [w563 _]
          tunnel: [w563 "Update"] -> w558
          frame Default {
          }
          frame "" {
          }
        }
      }
      frame "Back" {
        n244 = Unbundle By Name(w585) -> ("State"=w583:T2)
        n245 = case shown="\"Finished\"" w583 {
          tunnel: [OpenGDS_Installer_State."Init" ("State") OpenGDS_Installer_State."Init" ("State") OpenGDS_Installer_State."Options" ("State") OpenGDS_Installer_State."License" ("State") OpenGDS_Installer_State."Progress" ("State") OpenGDS_Installer_State."Cancelled" ("State") OpenGDS_Installer_State."Finished" ("State")] -> w582
          tunnel: [_ _ _ _ _ "Exit" "Exit"] -> w579
          frame "Init", Default {
          }
          frame "License" {
          }
          frame "Ready?" {
          }
          frame "Options" {
          }
          frame "Progress" {
          }
          frame "Cancelled" {
          }
          frame "Finished" {
          }
        }
        n246 = Bundle By Name(cluster=w585, "State"=w582) -> (w584:T3)
        n247 = case shown="Default" w579 {
          selector: w579 -> [w586 _]
          tunnel: [w586 "Update"] -> w581
          frame Default {
          }
          frame "" {
          }
        }
      }
    }
    n248 = Equal?(x=w157, y="Exit") -> (x = y?=w160:bool)
    n249 = Select(t="Abort", s=w156, f=w157) -> (s? t:f=w161:string)
  }
  n250 = Delete(path (use dialog)=w36, entire hierarchy (F)=TRUE) -> (error out=w33:errorcluster)  [unwired: 3 in, 2 out]
  n251 = stacked-sequence {
    tunnel: w34 -> [_]
    tunnel: w33 -> [_]
    frame #0 {
      n252 = invoke class="VI" method="FP.Close"() -> ()  [unwired: 3 in, 3 out]
    }
  }
  "Ready?-Text" <- "Click Install to begin the installation. \nClick Back to review or change any of your installation settings. \nClick Cancel to exit the Wizard." ("ProgressText")
